vi "test_PhotonPoseEstimator_ClosestToCamera.vi"(8 "error in (no error)":errorcluster) -> (0 "error out":errorcluster, 3 "Test Passed":bool)   [LabVIEW 2019]
uses:
  <vilib>/Rock Robotics/WPI/ThirdParty/PhotonVisionLib/TypeDef/PhotonEstimatedRobotPoseType.ctl
  <vilib>/Rock Robotics/WPI/ThirdParty/JAS_Junk/TrajLib/TypeDef/POSE3D.ctl
  <vilib>/Rock Robotics/WPI/ThirdParty/JAS_Junk/TrajLib/TypeDef/TRANSLATION3D.ctl
  <vilib>/Rock Robotics/WPI/ThirdParty/JAS_Junk/TrajLib/TypeDef/ROTATION3D.ctl
  <vilib>/Rock Robotics/WPI/ThirdParty/JAS_Junk/TrajLib/TypeDef/QUATERNION.ctl
  <vilib>/Rock Robotics/WPI/ThirdParty/PhotonVisionLib/TypeDef/PhotonTrackedTargetType.ctl
  <vilib>/Rock Robotics/WPI/ThirdParty/PhotonVisionLib/TypeDef/TargetCornerType.ctl
  <vilib>/Rock Robotics/WPI/ThirdParty/JAS_Junk/TrajLib/TypeDef/TRANSFORM3D.ctl
  <vilib>/Rock Robotics/WPI/ThirdParty/PhotonVisionLib/Enum/PhotonPoseStrategy_ENUM.ctl
  <vilib>/Rock Robotics/WPI/ThirdParty/JAS_Junk/TrajLib/VI/Quaternion_New.vi
  <vilib>/Rock Robotics/WPI/ThirdParty/PhotonVisionLib/SubVI/PhotonTargetModel_New_AprilTag36H11.vi
  <vilib>/Rock Robotics/WPI/ThirdParty/JAS_Junk/TrajLib/VI/TimeInterpRotation2d_New.vi
  <vilib>/Rock Robotics/WPI/ThirdParty/JAS_Junk/TrajLib/VI/Transform3d_Equals.vi
  <vilib>/Rock Robotics/WPI/ThirdParty/PhotonVisionLib/SubVI/PhotonPoseEstimator_SetCamera.vi
  <vilib>/Rock Robotics/WPI/ThirdParty/PhotonVisionLib/SubVI/PhotonPoseEstimator_SetRobotToCameraTransform.vi
  <vilib>/Rock Robotics/WPI/ThirdParty/PhotonVisionLib/SubVI/PhotonPoseEstimator_SetLastPose.vi
  <vilib>/Rock Robotics/WPI/ThirdParty/PhotonVisionLib/SubVI/PhotonEstimatedRobotPose_GetAll.vi
  <vilib>/Rock Robotics/WPI/ThirdParty/JAS_Junk/TrajLib/VI/Pose3d_ToPose2d.vi
  <vilib>/Rock Robotics/WPI/ThirdParty/PhotonVisionLib/SubVI/PhotonPoseEstimator_GetEmptyPose.vi
  <vilib>/Rock Robotics/WPI/ThirdParty/PhotonVisionLib/SubVI/PhotonPoseEstimator_EstimateClosestToCameraHeightPose.vi
  <vilib>/Rock Robotics/WPI/ThirdParty/PhotonVisionLib/SubVI/PhotonPipelineResult_GetTimeStampSecs.vi
  <vilib>/Rock Robotics/WPI/ThirdParty/PhotonVisionLib/SubVI/PhotonPoseEstimator_Update_All.vi
  <vilib>/Rock Robotics/WPI/ThirdParty/PhotonVisionLib/SubVI/PhotonTargetModel_New_RectPlanar.vi
  <vilib>/Rock Robotics/WPI/ThirdParty/JAS_Junk/TrajLib/Conv_Inches_Meters.vi
  <vilib>/Rock Robotics/WPI/ThirdParty/JAS_Junk/TrajLib/VI/Transform3d_GetTranslation3d.vi
  <vilib>/Rock Robotics/WPI/ThirdParty/JAS_Junk/TrajLib/VI/Transform3d_GetRotation3d.vi
  <vilib>/Rock Robotics/WPI/ThirdParty/JAS_Junk/TrajLib/VI/Rotation3d_Equals.vi
  <vilib>/Rock Robotics/WPI/ThirdParty/JAS_Junk/TrajLib/VI/Translation3d_Equals.vi
  <vilib>/Rock Robotics/WPI/ThirdParty/JAS_Junk/TrajLib/VI/Pose3d_getTranslation3d.vi
  <vilib>/Rock Robotics/WPI/ThirdParty/JAS_Junk/TrajLib/VI/Pose3d_getRotation3d.vi
  <vilib>/Rock Robotics/WPI/ThirdParty/JAS_Junk/TrajLib/VI/Translation3d_ToTranslation2d.vi
  <vilib>/Rock Robotics/WPI/ThirdParty/JAS_Junk/TrajLib/VI/Rotation3d_ToRotation2d.vi
  <vilib>/Rock Robotics/WPI/ThirdParty/JAS_Junk/TrajLib/Pose2d_New_TRRO.vi
  <vilib>/Rock Robotics/WPI/ThirdParty/JAS_Junk/TrajLib/VI/Rotation3d_Create_AxisAngle.vi
  <vilib>/Rock Robotics/WPI/ThirdParty/JAS_Junk/TrajLib/VI/Pose3d_New.vi
  <vilib>/Rock Robotics/WPI/ThirdParty/PhotonVisionLib/SubVI/PhotonPipelineResult_HasTargets.vi
  <vilib>/Rock Robotics/WPI/ThirdParty/PhotonVisionLib/SubVI/PhotonEstimatedRobotPose_New.vi
  <vilib>/Rock Robotics/WPI/ThirdParty/PhotonVisionLib/SubVI/PhotonPipelineResult_GetTargets.vi
  <vilib>/Rock Robotics/WPI/ThirdParty/JAS_Junk/TrajLib/VI/AprilTagFieldLayout_GetTagPose.vi
  <vilib>/Rock Robotics/WPI/ThirdParty/PhotonVisionLib/SubVI/PhotonTrackedTarget_GetFiducialId.vi
  <vilib>/Rock Robotics/WPI/ThirdParty/PhotonVisionLib/SubVI/PhotonPoseEstimator_Strategy_closestToCameraHeight_calc.vi
  <vilib>/Rock Robotics/WPI/ThirdParty/PhotonVisionLib/SubVI/PhotonTrackedTarget_GetAltCameraToTarget.vi
  <vilib>/Rock Robotics/WPI/ThirdParty/PhotonVisionLib/SubVI/PhotonTrackedTarget_GetBestCameraToTarget.vi
  <vilib>/Rock Robotics/WPI/ThirdParty/PhotonVisionLib/SubVI/PhotonTrackedTarget_GetPoseAmbiguity.vi
  <vilib>/Rock Robotics/WPI/ThirdParty/PhotonVisionLib/SubVI/PhotonPoseEstimator_GetFieldTags.vi
  <vilib>/Rock Robotics/WPI/ThirdParty/PhotonVisionLib/SubVI/PhotonPoseEstimator_GetRobotToCameraTransform.vi
  <vilib>/Rock Robotics/WPI/ThirdParty/PhotonVisionLib/SubVI/PhotonPoseEstimator_GetHighestAmbiguity.vi
  <vilib>/Rock Robotics/WPI/ThirdParty/PhotonVisionLib/SubVI/PhotonPoseEstimator_EstimateLowestAmbiguityPose.vi
  <vilib>/Rock Robotics/WPI/ThirdParty/PhotonVisionLib/SubVI/PhotonPoseEstimator_EstimateClosestToReferencePose.vi
  <vilib>/Rock Robotics/WPI/ThirdParty/PhotonVisionLib/SubVI/PhotonPoseEstimator_GetReferencePose.vi
  <vilib>/Rock Robotics/WPI/ThirdParty/PhotonVisionLib/SubVI/PhotonPoseEstimator_GetLastPose.vi
  <vilib>/Rock Robotics/WPI/ThirdParty/PhotonVisionLib/SubVI/PhotonPoseEstimator_SetReferencePose.vi
  <vilib>/Rock Robotics/WPI/ThirdParty/PhotonVisionLib/SubVI/PhotonPoseEstimator_EstimateClosestToLastPose.vi
  <vilib>/Rock Robotics/WPI/ThirdParty/PhotonVisionLib/SubVI/PhotonPoseEstimator_EstimateAverageBestTargetsPose.vi
  <vilib>/Rock Robotics/WPI/ThirdParty/PhotonVisionLib/SubVI/PhotonPoseEstimator_EstimateMultiTagOnCoprocPose.vi
  <vilib>/Rock Robotics/WPI/ThirdParty/PhotonVisionLib/SubVI/PhotonPoseEstimator_EstimatePnpDistanceTrigSolvePose.vi
  <vilib>/Rock Robotics/WPI/ThirdParty/PhotonVisionLib/SubVI/PhotonPoseEstimator_Strategy_constrainedPnpStrategy.vi
  <vilib>/Rock Robotics/WPI/ThirdParty/PhotonVisionLib/SubVI/PhotonTargetModel_New.vi
  <vilib>/Rock Robotics/WPI/ThirdParty/JAS_Junk/TrajLib/VI/Rotation3d_GetQuaterion.vi
  <vilib>/Rock Robotics/WPI/ThirdParty/JAS_Junk/TrajLib/VI/Quaternion_Equals.vi
  <vilib>/Rock Robotics/WPI/ThirdParty/JAS_Junk/TrajLib/Translation2d_Create.vi
  <vilib>/Rock Robotics/WPI/ThirdParty/JAS_Junk/TrajLib/Rotation2d_CreateAngle.vi
  <vilib>/Rock Robotics/WPI/ThirdParty/JAS_Junk/TrajLib/VI/Rotation3d_GetXYZ.vi
  <vilib>/Rock Robotics/WPI/ThirdParty/JAS_Junk/TrajLib/VI/Rotation3d_Create_Default.vi
  <vilib>/Rock Robotics/WPI/ThirdParty/JAS_Junk/TrajLib/VI/Vector_Norm.vi
  <vilib>/Rock Robotics/WPI/ThirdParty/JAS_Junk/TrajLib/VecBuilder_ArrayBy1Fill.vi
  <vilib>/Rock Robotics/WPI/ThirdParty/JAS_Junk/TrajLib/VI/Pose3d_New_Trans3dRot3d.vi
  <vilib>/Rock Robotics/WPI/ThirdParty/JAS_Junk/TrajLib/VI/AprilTag_GetAll.vi
  <vilib>/Rock Robotics/WPI/ThirdParty/JAS_Junk/TrajLib/VI/Pose3d_RelativeTo.vi
  <vilib>/Rock Robotics/WPI/ThirdParty/JAS_Junk/TrajLib/VI/Pose3d_TransformBy.vi
  <vilib>/Rock Robotics/WPI/ThirdParty/JAS_Junk/TrajLib/VI/Transform3d_Inverse.vi
  <vilib>/Rock Robotics/WPI/ThirdParty/JAS_Junk/TrajLib/VI/Transform3d_GetXYZ.vi
  <vilib>/Rock Robotics/WPI/ThirdParty/JAS_Junk/TrajLib/VI/Pose3d_getXYZ.vi
  <vilib>/Rock Robotics/WPI/ThirdParty/JAS_Junk/TrajLib/Transform2d_Create_TransRot.vi
  <vilib>/Rock Robotics/WPI/ThirdParty/PhotonVisionLib/SubVI/PhotonPoseEstimator_Strategy_closestToReferencePose_calc.vi
  <vilib>/Rock Robotics/WPI/ThirdParty/PhotonVisionLib/SubVI/PhotonPoseEstimator_Strategy_averageBestTargets_calc.vi
  <vilib>/Rock Robotics/WPI/ThirdParty/JAS_Junk/TrajLib/VI/Rotation3d_Plus.vi
  <vilib>/Rock Robotics/WPI/ThirdParty/JAS_Junk/TrajLib/VI/Translation3d_Plus.vi
  <vilib>/Rock Robotics/WPI/ThirdParty/JAS_Junk/TrajLib/VI/Translation3d_Times.vi
  <vilib>/Rock Robotics/WPI/ThirdParty/JAS_Junk/TrajLib/VI/Rotation3d_Times.vi
  <vilib>/Rock Robotics/WPI/ThirdParty/JAS_Junk/TrajLib/VI/Translation3d_Create_Default.vi
  <vilib>/Rock Robotics/WPI/ThirdParty/JAS_Junk/TrajLib/VI/Pose3d_New_Default.vi
  <vilib>/Rock Robotics/WPI/ThirdParty/JAS_Junk/TrajLib/VI/Pose3d_Plus.vi
  <vilib>/Rock Robotics/WPI/ThirdParty/JAS_Junk/TrajLib/VI/AprilTagFieldLayout_GetOriginPosition.vi
  <vilib>/Rock Robotics/WPI/ThirdParty/PhotonVisionLib/SubVI/PhotonPipelineResult_GetMultiTagResult.vi
  <vilib>/Rock Robotics/WPI/ThirdParty/PhotonVisionLib/SubVI/PhotonPipelineResult_GetBestTarget.vi
  <vilib>/Rock Robotics/WPI/ThirdParty/PhotonVisionLib/SubVI/PhotonTrackedTarget_GetPitch.vi
  <vilib>/Rock Robotics/WPI/ThirdParty/PhotonVisionLib/SubVI/PhotonTrackedTarget_GetYaw.vi
  <vilib>/Rock Robotics/WPI/ThirdParty/JAS_Junk/TrajLib/Units_DegreesToRadians.vi
  <vilib>/Rock Robotics/WPI/ThirdParty/JAS_Junk/TrajLib/VI/Translation3d_GetNorm.vi
  <vilib>/Rock Robotics/WPI/ThirdParty/JAS_Junk/TrajLib/VI/Translation3d_Create_DistAng.vi
  <vilib>/Rock Robotics/WPI/ThirdParty/JAS_Junk/TrajLib/VI/Translation3d_RotateBy.vi
  <vilib>/Rock Robotics/WPI/ThirdParty/JAS_Junk/TrajLib/Translation2d_RotateBy.vi
  <vilib>/Rock Robotics/WPI/ThirdParty/JAS_Junk/TrajLib/Pose2d_getTranslation.vi
  <vilib>/Rock Robotics/WPI/ThirdParty/JAS_Junk/TrajLib/Translation2d_Plus.vi
  <vilib>/Rock Robotics/WPI/ThirdParty/JAS_Junk/TrajLib/Translation2d_UnaryMinus.vi
  <vilib>/Rock Robotics/WPI/ThirdParty/JAS_Junk/TrajLib/VI/Pose3d_New_Pose2d.vi
  <vilib>/Rock Robotics/WPI/ThirdParty/JAS_Junk/TrajLib/VI/TimeInterpRotation2d_GetSample.vi
  <vilib>/Rock Robotics/WPI/ThirdParty/PhotonVisionLib/SubVI/PhotonPoseEstimator_GetHeadingBuffer.vi
  <vilib>/Rock Robotics/WPI/ThirdParty/JAS_Junk/TrajLib/VI/Quaternion_Get_Vect.vi
  <vilib>/Rock Robotics/WPI/ThirdParty/JAS_Junk/TrajLib/VI/Quaternion_Get_W.vi
  <vilib>/Rock Robotics/WPI/ThirdParty/JAS_Junk/TrajLib/VI/Quaternion_Get_All.vi
  <vilib>/Rock Robotics/WPI/ThirdParty/JAS_Junk/TrajLib/VI/Quaternion_New_Default.vi
  <vilib>/Rock Robotics/WPI/ThirdParty/JAS_Junk/TrajLib/MatBuilder_Create.vi
  <vilib>/Rock Robotics/WPI/ThirdParty/JAS_Junk/TrajLib/VI/Transform3d_Create_Pose3dPose3d.vi
  <vilib>/Rock Robotics/WPI/ThirdParty/JAS_Junk/TrajLib/VI/Rotation3d_UnaryMinus.vi
  <vilib>/Rock Robotics/WPI/ThirdParty/JAS_Junk/TrajLib/VI/Translation3d_UnaryMinus.vi
  <vilib>/Rock Robotics/WPI/ThirdParty/JAS_Junk/TrajLib/VI/Translation3d_GetXYZ.vi
  <vilib>/Rock Robotics/WPI/ThirdParty/PhotonVisionLib/SubVI/PhotonPoseEstimator_CalcDifference.vi
  <vilib>/Rock Robotics/WPI/ThirdParty/JAS_Junk/TrajLib/VI/Rotation3d_RotateBy.vi
  <vilib>/Rock Robotics/WPI/ThirdParty/JAS_Junk/TrajLib/Conv_Deg_Radians.vi
  <vilib>/Rock Robotics/WPI/ThirdParty/JAS_Junk/TrajLib/VI/Quaternion_Times.vi
  <vilib>/Rock Robotics/WPI/ThirdParty/JAS_Junk/TrajLib/VI/Quaternion_Inverse.vi
  <vilib>/Rock Robotics/WPI/ThirdParty/JAS_Junk/TrajLib/Pose2d_getXYAngle.vi
  <vilib>/Rock Robotics/WPI/ThirdParty/JAS_Junk/TrajLib/Rotation2d_Interpolate.vi
  <vilib>/Rock Robotics/WPI/ThirdParty/JAS_Junk/TrajLib/VI/Translation3d_Minus.vi
  <vilib>/Rock Robotics/WPI/ThirdParty/JAS_Junk/TrajLib/VI/Rotation3d_Minus.vi
  <vilib>/Rock Robotics/WPI/ThirdParty/JAS_Junk/TrajLib/VI/Rotation3d_Create_Quaternion.vi
  <vilib>/Rock Robotics/WPI/ThirdParty/JAS_Junk/TrajLib/VI/Translation3d_GetDistance.vi
  <vilib>/Rock Robotics/WPI/ThirdParty/JAS_Junk/TrajLib/Rotation2d_Plus.vi
  <vilib>/Rock Robotics/WPI/ThirdParty/JAS_Junk/TrajLib/Rotation2d_Minus.vi
  <vilib>/Rock Robotics/WPI/ThirdParty/JAS_Junk/TrajLib/MathUtil_Clamp.vi
  <vilib>/Rock Robotics/WPI/ThirdParty/JAS_Junk/TrajLib/Rotation2d_Times.vi
  <vilib>/Rock Robotics/WPI/ThirdParty/JAS_Junk/TrajLib/VI/Quaternion_Normalize.vi
  <vilib>/Rock Robotics/WPI/ThirdParty/JAS_Junk/TrajLib/Rotation2d_RotateBy.vi
  <vilib>/Rock Robotics/WPI/ThirdParty/JAS_Junk/TrajLib/Rotation2d_UnaryMinus.vi
  <vilib>/Rock Robotics/WPI/ThirdParty/JAS_Junk/TrajLib/Rotation2d_CreateXY.vi
  <vilib>/Rock Robotics/WPI/ThirdParty/JAS_Junk/TrajLib/Util_CalcDist.vi
  <vilib>/Rock Robotics/WPI/ThirdParty/PhotonVisionLib/SubVI/PhotonVision_Globals.vi
  <vilib>/gmath/interp.llb/Search Ordered Table.vi
  <vilib>/Rock Robotics/WPI/ThirdParty/JAS_Junk/TrajLib/Trajectory_Library.lvlib
  <vilib>/Rock Robotics/WPI/ThirdParty/PhotonVisionLib/PhotonVisionLib.lvlib
panel:
  out "Test 2 Passed":bool
  out "Test 1 Passed":bool
  out "Pos Found":bool
  out "PhotonEstimatedRobotPose":T1={"EstimatedPose"={"Translation3d"={"X"=0.0, "Y"=0.0, "Z"=0.0}, "Rotation3d"={"Q_quaternion"={"R"=1.0, "V"=[0.0, 0.0, 0.0]}}}, "TimeStamp_Seconds"=0.0, "targetsUsed"=[], "Strategy"=enum."LOWEST_AMBIGUITY"} {"targetsUsed"."AltCameraToTarget"."TRANSLATION3D"."Z" format="%14.3f"; "targetsUsed"."AltCameraToTarget"."TRANSLATION3D"."Y" format="%14.3f"; "targetsUsed"."AltCameraToTarget"."TRANSLATION3D"."X" format="%14.3f"; "targetsUsed"."BestCameraToTarget"."TRANSLATION3D"."Z" format="%14.3f"; "targetsUsed"."BestCameraToTarget"."TRANSLATION3D"."Y" format="%14.3f"; "targetsUsed"."BestCameraToTarget"."TRANSLATION3D"."X" format="%14.3f"; "EstimatedPose"."Translation3d"."Z" format="%14.3f"; "EstimatedPose"."Translation3d"."Y" format="%14.3f"; "EstimatedPose"."Translation3d"."X" format="%14.3f"}
  out "Test 0 Passed":bool
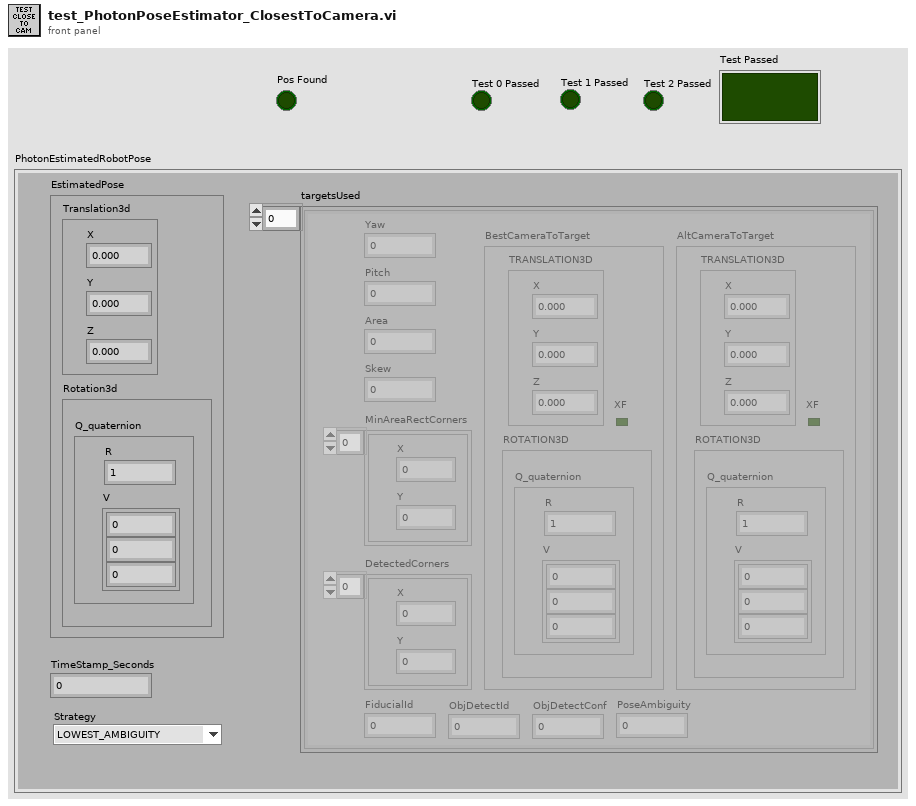
[diagram p1: front panel]
types:
  T1 = typedef "PhotonVisionLib.lvlib/PhotonEstimatedRobotPoseType.ctl" = cluster{"EstimatedPose":T2, "TimeStamp_Seconds":dbl, "targetsUsed":T6[], "Strategy":T9}
  T2 = typedef "Trajectory_Library.lvlib/POSE3D.ctl" = cluster{"Translation3d":T3, "Rotation3d":T4}
  T3 = typedef "Trajectory_Library.lvlib/TRANSLATION3D.ctl" = cluster{"X":dbl, "Y":dbl, "Z":dbl}
  T4 = typedef "Trajectory_Library.lvlib/ROTATION3D.ctl" = cluster{"Q_quaternion":T5}
  T5 = typedef "Trajectory_Library.lvlib/QUATERNION.ctl" = cluster{"R":dbl, "V":dbl[]}
  T6 = typedef "PhotonVisionLib.lvlib/PhotonTrackedTargetType.ctl" = cluster{"Yaw":dbl, "Pitch":dbl, "Area":dbl, "Skew":dbl, "MinAreaRectCorners":T7[], "BestCameraToTarget":T8, "FiducialId":i32, "AltCameraToTarget":T8, "PoseAmbiguity":dbl, "DetectedCorners":T7[], "ObjDetectId":i32, "ObjDetectConf":sgl}
  T7 = typedef "PhotonVisionLib.lvlib/TargetCornerType.ctl" = cluster{"X":dbl, "Y":dbl}
  T8 = typedef "Trajectory_Library.lvlib/TRANSFORM3D.ctl" = cluster{"TRANSLATION3D":T3, "ROTATION3D":T4, "XF":bool}
  T9 = typedef "PhotonVisionLib.lvlib/PhotonPoseStrategy_ENUM.ctl" = enum16{"LOWEST_AMBIGUITY", "CLOSEST_TO_CAMERA_HEIGHT", "CLOSEST_TO_REFERENCE_POSE", "CLOSEST_TO_LAST_POSE", "AVERAGE_BEST_TARGETS", "MULTI_TAG_PNP_ON_COPROCESSOR", "MULTI_TAG_PNP_ON_RIO", "PNP_DISTANCE_TRIG_SOLVE", "CONSTRAINED_SOLVEPNP"}
  T10 = typedef "Trajectory_Library.lvlib/AprilTagFieldLayout.ctl" = cluster{"AprilTagMap":map{i32, T11}, "FieldLength":dbl, "FieldWidth":dbl, "OriginPosition ":T12, "OriginPose3d":T2}
  T11 = typedef "Trajectory_Library.lvlib/AprilTag.ctl" = cluster{"ID":i32, "POSE3D":T2}
  T12 = typedef "Trajectory_Library.lvlib/AprilTagFieldLayoutOrignPosition_ENUM.ctl" = enum16{"kBlueAllianceWallRightSide,", "kRedAllianceWallRightSide,"}
  T13 = typedef "PhotonVisionLib.lvlib/PhotonPipelineMetadataType.ctl" = cluster{"CaptureTimestampMicros":i64, "PublishTimestampMicros":i64, "SequenceID":i64, "TimeSinceLastPong":i64}
  T14 = typedef "PhotonVisionLib.lvlib/PhotonPipelineResultType.ctl" = cluster{"Targets":T6[], "PhotonMultiTargetPNPResult":T15, "PhotonPipelineMetadata":T13}
  T15 = typedef "PhotonVisionLib.lvlib/PhotonMultiTargetPNPResultType.ctl" = cluster{"PhotonPNPResult":T16, "FiducialIDsUsed":i16[]}
  T16 = typedef "PhotonVisionLib.lvlib/PhotonPNPResultType.ctl" = cluster{"IsPresent":bool, "bestReprojErr":dbl, "altReprojErr":dbl, "ambiguity":dbl, "Best":T8, "Alt":T8}
  T17 = typedef "PhotonVisionLib.lvlib/PhotonPoseEstimator_Configuration.ctl" = cluster{"Primary Strategy":T9, "Camera":string, "Initial Pose":T2, "HighestAmbiguity":dbl, "RobotToCamera":T8, "FallBack Strategy":T9, "BaseNTName":string}
  T18 = typedef "PhotonVisionLib.lvlib/PhotonPoseEstimatorType.ctl" = cluster{"LastPose":T2, "ReferencePose":T2, "FieldTags":T10, "PrimaryStratety":T9, "Camera":string, "RobotToCamera":T8, "ReportedErrors":dbl[], "HighestAmbiguity":dbl, "MultiTagFallbackStrategy":T9, "PoseCacheTimeoutSec":dbl, "PhotonTargetModel":T19, "BaseNTName":string}
  T19 = typedef "PhotonVisionLib.lvlib/PhotonTargetModel.ctl" = cluster{"Vertices":T3[], "IsPlaner":bool, "IsSpherical":bool}
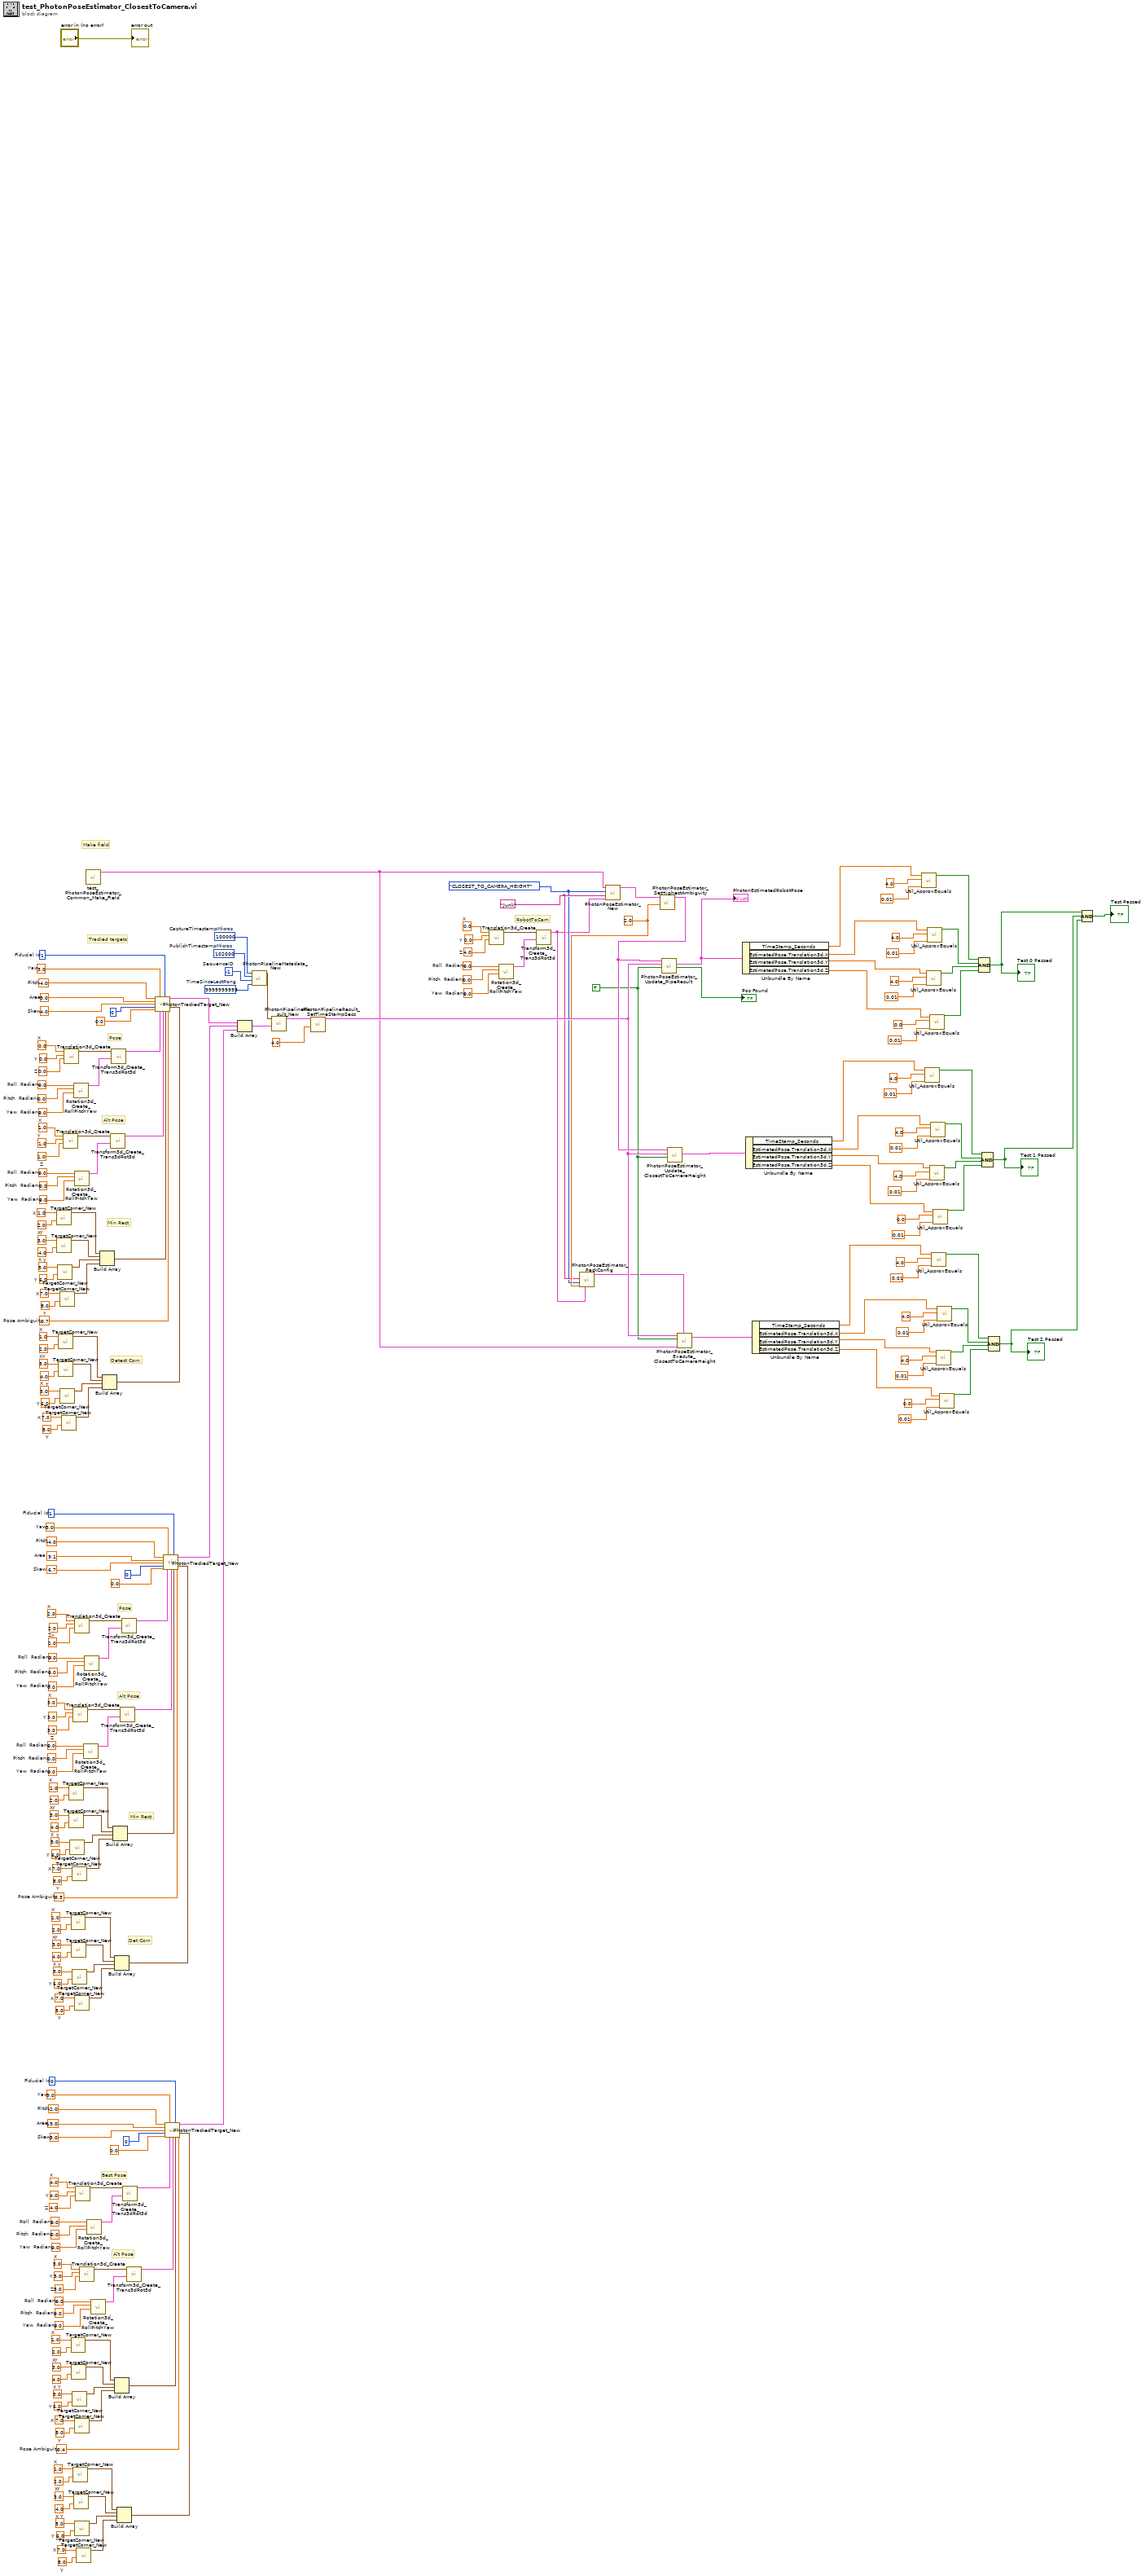
[diagram p0: block diagram]
diagram:
  w6 = 2.0 ("HighestAmbiguity")
  w54 = i64 100000  # CaptureTimestampMicros
  w55 = i64 102000  # PublishTimestampMicros
  w56 = i64 -1  # SequenceID
  w57 = i64 9999999999  # TimeSinceLastPong
  w43 = TRUE ("Has Results")
  w68 = 0.0  # Roll  Radians
  w67 = 0.0  # Pitch  Radians
  w66 = 0.0  # Yaw  Radians
  w71 = 4.0  # Z
  w70 = 0.0  # X
  w69 = 0.0  # Y
  w5 = "Junk" ("Camera")
  w4 = PhotonPoseStrategy_ENUM."CLOSEST_TO_CAMERA_HEIGHT" ("Strategy")
  w93 = 0.0  # Roll  Radians
  w92 = 0.0  # Pitch  Radians
  w91 = 0.0  # Yaw  Radians
  w96 = 4.0  # Z
  w95 = 4.0  # X
  w94 = 4.0  # Y
  w101 = 0.0  # Roll  Radians
  w100 = 0.0  # Pitch  Radians
  w99 = 0.0  # Yaw  Radians
  w104 = 5.0  # Z
  w103 = 5.0  # X
  w102 = 5.0  # Y
  w111 = 7.0  # X
  w112 = 8.0  # Y
  w113 = 5.0  # X
  w114 = 6.0  # Y
  w115 = 3.0  # X
  w116 = 4.0  # Y
  w117 = 1.0  # X
  w118 = 2.0  # Y
  w123 = 7.0  # X
  w124 = 8.0  # Y
  w125 = 5.0  # X
  w126 = 6.0  # Y
  w127 = 3.0  # X
  w128 = 4.0  # Y
  w129 = 1.0  # X
  w130 = 2.0  # Y
  w131 = -2.0  # Pitch
  w132 = 19.0  # Area
  w133 = 3.0  # Skew
  w134 = 0  # Fiducial Id
  w135 = 0.4  # Pose Ambiguity
  w136 = 9.0  # Yaw
  w143 = 0.0  # Roll  Radians
  w142 = 0.0  # Pitch  Radians
  w141 = 0.0  # Yaw  Radians
  w146 = 2.0  # Z
  w145 = 2.0  # X
  w144 = 2.0  # Y
  w151 = 0.0  # Roll  Radians
  w150 = 0.0  # Pitch  Radians
  w149 = 0.0  # Yaw  Radians
  w154 = 3.0  # Z
  w153 = 3.0  # X
  w152 = 3.0  # Y
  w161 = 7.0  # X
  w162 = 8.0  # Y
  w163 = 5.0  # X
  w164 = 6.0  # Y
  w165 = 3.0  # X
  w166 = 4.0  # Y
  w167 = 1.0  # X
  w168 = 2.0  # Y
  w173 = 7.0  # X
  w174 = 8.0  # Y
  w175 = 5.0  # X
  w176 = 6.0  # Y
  w177 = 3.0  # X
  w178 = 4.0  # Y
  w179 = 1.0  # X
  w180 = 2.0  # Y
  w181 = -4.0  # Pitch
  w182 = 9.1  # Area
  w183 = 6.7  # Skew
  w184 = 1  # Fiducial Id
  w185 = 0.3  # Pose Ambiguity
  w186 = 3.0  # Yaw
  w193 = 0.0  # Roll  Radians
  w192 = 0.0  # Pitch  Radians
  w191 = 0.0  # Yaw  Radians
  w196 = 0.0  # Z
  w195 = 0.0  # X
  w194 = 0.0  # Y
  w201 = 0.0  # Roll  Radians
  w200 = 0.0  # Pitch  Radians
  w199 = 0.0  # Yaw  Radians
  w204 = 1.0  # Z
  w203 = 1.0  # X
  w202 = 1.0  # Y
  w211 = 7.0  # X
  w212 = 8.0  # Y
  w213 = 5.0  # X
  w214 = 6.0  # Y
  w215 = 3.0  # X
  w216 = 4.0  # Y
  w217 = 1.0  # X
  w218 = 2.0  # Y
  w223 = 7.0  # X
  w224 = 8.0  # Y
  w225 = 5.0  # X
  w226 = 6.0  # Y
  w227 = 3.0  # X
  w228 = 4.0  # Y
  w229 = 1.0  # X
  w230 = 2.0  # Y
  w231 = -4.0  # Pitch
  w232 = 9.0  # Area
  w233 = 4.0  # Skew
  w234 = 1  # Fiducial Id
  w235 = 0.7  # Pose Ambiguity
  w236 = 3.0  # Yaw
  # "RobotToCam"
  # "Det Corn"
  # "Min Rect"
  # "Pose"
  # "Detect Corn"
  # "Min Rect"
  # "Tracked targets"
  # "Make field"
  # "Best Pose"
  # "Alt Pose"
  # "Alt Pose"
  # "Pose"
  # "Alt Pose"
  n1 = call <vilib>:"TargetCorner_New.vi"("Y"=w230, "X"=w229) -> ("TargetCorner"=w222:T7)  [unwired: 9 in]
  n2 = call <vilib>:"TargetCorner_New.vi"("Y"=w228, "X"=w227) -> ("TargetCorner"=w221:T7)  [unwired: 9 in]
  n3 = call <vilib>:"TargetCorner_New.vi"("Y"=w226, "X"=w225) -> ("TargetCorner"=w220:T7)  [unwired: 9 in]
  n4 = call <vilib>:"TargetCorner_New.vi"("Y"=w218, "X"=w217) -> ("TargetCorner"=w210:T7)  [unwired: 9 in]
  n5 = call <vilib>:"TargetCorner_New.vi"("Y"=w216, "X"=w215) -> ("TargetCorner"=w209:T7)  [unwired: 9 in]
  n6 = call <vilib>:"TargetCorner_New.vi"("Y"=w224, "X"=w223) -> ("TargetCorner"=w219:T7)  [unwired: 9 in]
  n7 = call <vilib>:"TargetCorner_New.vi"("Y"=w214, "X"=w213) -> ("TargetCorner"=w208:T7)  [unwired: 9 in]
  n8 = call <vilib>:"TargetCorner_New.vi"("Y"=w212, "X"=w211) -> ("TargetCorner"=w207:T7)  [unwired: 9 in]
  n9 = call <vilib>:"Translation3d_Create.vi"("Z"=w204, "Y"=w202, "X"=w203) -> ("TRANSLATION3D"=w198:T3)  [unwired: 8 in]
  n10 = call <vilib>:"Translation3d_Create.vi"("Z"=w196, "Y"=w194, "X"=w195) -> ("TRANSLATION3D"=w190:T3)  [unwired: 8 in]
  n11 = call <vilib>:"TargetCorner_New.vi"("Y"=w180, "X"=w179) -> ("TargetCorner"=w172:T7)  [unwired: 9 in]
  n12 = call <vilib>:"TargetCorner_New.vi"("Y"=w178, "X"=w177) -> ("TargetCorner"=w171:T7)  [unwired: 9 in]
  n13 = call <vilib>:"TargetCorner_New.vi"("Y"=w176, "X"=w175) -> ("TargetCorner"=w170:T7)  [unwired: 9 in]
  n14 = call <vilib>:"TargetCorner_New.vi"("Y"=w168, "X"=w167) -> ("TargetCorner"=w160:T7)  [unwired: 9 in]
  n15 = call <vilib>:"TargetCorner_New.vi"("Y"=w130, "X"=w129) -> ("TargetCorner"=w122:T7)  [unwired: 9 in]
  n16 = call <vilib>:"TargetCorner_New.vi"("Y"=w166, "X"=w165) -> ("TargetCorner"=w159:T7)  [unwired: 9 in]
  n17 = call <vilib>:"TargetCorner_New.vi"("Y"=w128, "X"=w127) -> ("TargetCorner"=w121:T7)  [unwired: 9 in]
  n18 = call <vilib>:"TargetCorner_New.vi"("Y"=w174, "X"=w173) -> ("TargetCorner"=w169:T7)  [unwired: 9 in]
  n19 = call <vilib>:"TargetCorner_New.vi"("Y"=w164, "X"=w163) -> ("TargetCorner"=w158:T7)  [unwired: 9 in]
  n20 = call <vilib>:"TargetCorner_New.vi"("Y"=w126, "X"=w125) -> ("TargetCorner"=w120:T7)  [unwired: 9 in]
  n21 = call <vilib>:"Translation3d_Create.vi"("Z"=w154, "Y"=w152, "X"=w153) -> ("TRANSLATION3D"=w148:T3)  [unwired: 8 in]
  n22 = call <vilib>:"TargetCorner_New.vi"("Y"=w118, "X"=w117) -> ("TargetCorner"=w110:T7)  [unwired: 9 in]
  n23 = call <vilib>:"Rotation3d_Create_RollPitchYaw.vi"("Yaw"=w191, "Pitch"=w192, "Roll"=w193) -> ("Rotation3d"=w189:T4)  [unwired: 8 in]
  n24 = call <vilib>:"TargetCorner_New.vi"("Y"=w116, "X"=w115) -> ("TargetCorner"=w109:T7)  [unwired: 9 in]
  n25 = call <vilib>:"Rotation3d_Create_RollPitchYaw.vi"("Yaw"=w199, "Pitch"=w200, "Roll"=w201) -> ("Rotation3d"=w197:T4)  [unwired: 8 in]
  n26 = call <vilib>:"Translation3d_Create.vi"("Z"=w146, "Y"=w144, "X"=w145) -> ("TRANSLATION3D"=w140:T3)  [unwired: 8 in]
  n27 = call <vilib>:"TargetCorner_New.vi"("Y"=w162, "X"=w161) -> ("TargetCorner"=w157:T7)  [unwired: 9 in]
  n28 = call <vilib>:"TargetCorner_New.vi"("Y"=w124, "X"=w123) -> ("TargetCorner"=w119:T7)  [unwired: 9 in]
  n29 = call <vilib>:"TargetCorner_New.vi"("Y"=w114, "X"=w113) -> ("TargetCorner"=w108:T7)  [unwired: 9 in]
  n30 = call <vilib>:"Translation3d_Create.vi"("Z"=w96, "Y"=w94, "X"=w95) -> ("TRANSLATION3D"=w90:T3)  [unwired: 8 in]
  n31 = call <vilib>:"TargetCorner_New.vi"("Y"=w112, "X"=w111) -> ("TargetCorner"=w107:T7)  [unwired: 9 in]
  n32 = call <vilib>:"Translation3d_Create.vi"("Z"=w104, "Y"=w102, "X"=w103) -> ("TRANSLATION3D"=w98:T3)  [unwired: 8 in]
  n33 = call <vilib>:"Rotation3d_Create_RollPitchYaw.vi"("Yaw"=w149, "Pitch"=w150, "Roll"=w151) -> ("Rotation3d"=w147:T4)  [unwired: 8 in]
  n34 = call <vilib>:"Rotation3d_Create_RollPitchYaw.vi"("Yaw"=w141, "Pitch"=w142, "Roll"=w143) -> ("Rotation3d"=w139:T4)  [unwired: 8 in]
  n35 = call "test_PhotonPoseEstimator_Common_Make_Field.vi"() -> ("AprilTagFieldLayout"=w42:T10)  [unwired: 11 in]
  n36 = call <vilib>:"Rotation3d_Create_RollPitchYaw.vi"("Yaw"=w91, "Pitch"=w92, "Roll"=w93) -> ("Rotation3d"=w89:T4)  [unwired: 8 in]
  n37 = call <vilib>:"Rotation3d_Create_RollPitchYaw.vi"("Yaw"=w99, "Pitch"=w100, "Roll"=w101) -> ("Rotation3d"=w97:T4)  [unwired: 8 in]
  n38 = Build Array(w222, w221, w220, w219) -> (w206:T7[])
  n39 = Build Array(w210, w209, w208, w207) -> (w205:T7[])
  n40 = call <vilib>:"Transform3d_Create_Trans3dRot3d.vi"("Rotation3d"=w197, "Translation3d"=w198) -> ("Transform3d"=w187:T8)  [unwired: 9 in]
  n41 = call <vilib>:"Transform3d_Create_Trans3dRot3d.vi"("Rotation3d"=w189, "Translation3d"=w190) -> ("Transform3d"=w188:T8)  [unwired: 9 in]
  n42 = Build Array(w172, w171, w170, w169) -> (w156:T7[])
  n43 = Build Array(w160, w159, w158, w157) -> (w155:T7[])
  n44 = Build Array(w122, w121, w120, w119) -> (w106:T7[])
  n45 = Build Array(w110, w109, w108, w107) -> (w105:T7[])
  n46 = call <vilib>:"Transform3d_Create_Trans3dRot3d.vi"("Rotation3d"=w147, "Translation3d"=w148) -> ("Transform3d"=w137:T8)  [unwired: 9 in]
  n47 = call <vilib>:"Transform3d_Create_Trans3dRot3d.vi"("Rotation3d"=w139, "Translation3d"=w140) -> ("Transform3d"=w138:T8)  [unwired: 9 in]
  n48 = call <vilib>:"Transform3d_Create_Trans3dRot3d.vi"("Rotation3d"=w89, "Translation3d"=w90) -> ("Transform3d"=w88:T8)  [unwired: 9 in]
  n49 = call <vilib>:"Transform3d_Create_Trans3dRot3d.vi"("Rotation3d"=w97, "Translation3d"=w98) -> ("Transform3d"=w87:T8)  [unwired: 9 in]
  n50 = call <vilib>:"PhotonTrackedTarget_New.vi"("Pitch"=w231, "Yaw"=w236, "Fiducial Id"=w234, "Area"=w232, "Skew"=w233, "ObjDetectId"=0, "DetectedCorners"=w205, "DetectObjConf"=sgl 0.0, "BestCameraToTarget"=w188, "AltCameraToTarget"=w187, "MinAreaRectCorners"=w206, "Pose Ambiguity"=w235) -> ("TrackedTarget"=w86:T6)  [unwired: 3 in]
  n51 = call <vilib>:"PhotonTrackedTarget_New.vi"("Pitch"=w181, "Yaw"=w186, "Fiducial Id"=w184, "Area"=w182, "Skew"=w183, "ObjDetectId"=0, "DetectedCorners"=w155, "DetectObjConf"=sgl 0.0, "BestCameraToTarget"=w138, "AltCameraToTarget"=w137, "MinAreaRectCorners"=w156, "Pose Ambiguity"=w185) -> ("TrackedTarget"=w85:T6)  [unwired: 3 in]
  n52 = call <vilib>:"PhotonTrackedTarget_New.vi"("Pitch"=w131, "Yaw"=w136, "Fiducial Id"=w134, "Area"=w132, "Skew"=w133, "ObjDetectId"=0, "DetectedCorners"=w105, "DetectObjConf"=sgl 0.0, "BestCameraToTarget"=w88, "AltCameraToTarget"=w87, "MinAreaRectCorners"=w106, "Pose Ambiguity"=w135) -> ("TrackedTarget"=w84:T6)  [unwired: 3 in]
  n53 = Build Array(w86, w85, w84) -> (w83:T6[])
  n54 = call <vilib>:"PhotonPipelineMetadata_New.vi"("TimeSinceLastPong"=w57, "SequenceID"=w56, "PublishTimestampMicros"=w55, "CaptureTimestampMicros"=w54) -> ("PhotonPipelineMetadata"=w53:T13)  [unwired: 7 in]
  n55 = call <vilib>:"PhotonPipelineResult_New.vi"("TrackedTargets"=w83, "Metadata"=w53) -> ("PhotonPipelineResult"=w82:T14)  [unwired: 9 in]
  n56 = call <vilib>:"PhotonPipelineResult_SetTimeStampSecs.vi"("TimeStampSec"=4.0, "PhotonPipelineResult"=w82) -> ("Out PhotonPipelineResult"=w44:T14)  [unwired: 9 in]
  n57 = call <vilib>:"Translation3d_Create.vi"("Z"=w71, "Y"=w69, "X"=w70) -> ("TRANSLATION3D"=w65:T3)  [unwired: 8 in]
  n58 = call <vilib>:"Rotation3d_Create_RollPitchYaw.vi"("Yaw"=w66, "Pitch"=w67, "Roll"=w68) -> ("Rotation3d"=w64:T4)  [unwired: 8 in]
  n59 = call <vilib>:"Transform3d_Create_Trans3dRot3d.vi"("Rotation3d"=w64, "Translation3d"=w65) -> ("Transform3d"=w3:T8)  [unwired: 9 in]
  n60 = call <vilib>:"PhotonPoseEstimator_PackConfig.vi"("RobotToCamera"=w3, "HighestAmbiguity"=w6, "PirmaryStrategy"=w4, "Camera"=w5) -> ("PoseEstimator_Configuration"=w7:T17)  [unwired: 7 in]
  n61 = call <vilib>:"PhotonPoseEstimator_New.vi"("RobotToCamera"=w3, "Camera"=w5, "Strategy"=w4, "AprilTagFieldLayout"=w42) -> ("PhotonPoseEstimator"=w46:T18)  [unwired: 7 in]
  n62 = call <vilib>:"PhotonPoseEstimator_SetHighestAmbiguity.vi"("HighestAmbiguity"=w6, "PhotonPoseEstimator"=w46) -> ("out PhotonPoseEstimator"=w45:T18)  [unwired: 9 in]
  n63 = call <vilib>:"PhotonPoseEstimator_Update_PipeResult.vi"("Has Results"=w43, "PipelineResult"=w44, "PhotonPoseEstimator"=w45) -> ("Pos Found"=→"Pos Found":bool, "PhotonEstimatedRobotPose"=w59:T1)  [unwired: 6 in, 1 out]
  "PhotonEstimatedRobotPose" <- w59
  n64 = call <vilib>:"PhotonPoseEstimator_Update_ClosestToCameraHeight.vi"("Has Results"=w43, "PipelineResult"=w44, "PhotonPoseEstimator"=w45) -> ("PhotonEstimatedRobotPose"=w25:T1)  [unwired: 6 in, 2 out]
  n65 = call <vilib>:"PhotonPoseEstimator_Execute_ClosestToCameraHeight.vi"("Configuration"=w7, "AprilTagFieldLayout"=w42, "PIpeline Has \nNew Results"=w43, "PipelineResult"=w44) -> ("PhotonEstimatedRobotPose"=w8:T1)  [unwired: 2 in, 5 out]
  n66 = Unbundle By Name(w59) -> ("TimeStamp_Seconds"=w60:dbl, "EstimatedPose.Translation3d.X"=w74:dbl, "EstimatedPose.Translation3d.Y"=w73:dbl, "EstimatedPose.Translation3d.Z"=w72:dbl)
  n67 = Unbundle By Name(w25) -> ("TimeStamp_Seconds"=w26:dbl, "EstimatedPose.Translation3d.X"=w32:dbl, "EstimatedPose.Translation3d.Y"=w31:dbl, "EstimatedPose.Translation3d.Z"=w30:dbl)
  n68 = Unbundle By Name(w8) -> ("TimeStamp_Seconds"=w9:dbl, "EstimatedPose.Translation3d.X"=w15:dbl, "EstimatedPose.Translation3d.Y"=w14:dbl, "EstimatedPose.Translation3d.Z"=w13:dbl)
  n69 = call <vilib>:"Util_ApproxEquals.vi"("Tolerance"=0.01, "Value 2"=4.0, "Value 1"=w60) -> ("ApproxEquals"=w61:bool)  [unwired: 8 in]
  n70 = call <vilib>:"Util_ApproxEquals.vi"("Tolerance"=0.01, "Value 2"=4.0, "Value 1"=w26) -> ("ApproxEquals"=w27:bool)  [unwired: 8 in]
  n71 = call <vilib>:"Util_ApproxEquals.vi"("Tolerance"=0.01, "Value 2"=4.0, "Value 1"=w73) -> ("ApproxEquals"=w76:bool)  [unwired: 8 in]
  n72 = call <vilib>:"Util_ApproxEquals.vi"("Tolerance"=0.01, "Value 2"=4.0, "Value 1"=w74) -> ("ApproxEquals"=w239:bool)  [unwired: 8 in]
  n73 = call <vilib>:"Util_ApproxEquals.vi"("Tolerance"=0.01, "Value 2"=0.0, "Value 1"=w72) -> ("ApproxEquals"=w75:bool)  [unwired: 8 in]
  n74 = call <vilib>:"Util_ApproxEquals.vi"("Tolerance"=0.01, "Value 2"=4.0, "Value 1"=w31) -> ("ApproxEquals"=w34:bool)  [unwired: 8 in]
  n75 = call <vilib>:"Util_ApproxEquals.vi"("Tolerance"=0.01, "Value 2"=4.0, "Value 1"=w32) -> ("ApproxEquals"=w39:bool)  [unwired: 8 in]
  n76 = call <vilib>:"Util_ApproxEquals.vi"("Tolerance"=0.01, "Value 2"=4.0, "Value 1"=w9) -> ("ApproxEquals"=w10:bool)  [unwired: 8 in]
  n77 = call <vilib>:"Util_ApproxEquals.vi"("Tolerance"=0.01, "Value 2"=0.0, "Value 1"=w30) -> ("ApproxEquals"=w33:bool)  [unwired: 8 in]
  n78 = call <vilib>:"Util_ApproxEquals.vi"("Tolerance"=0.01, "Value 2"=4.0, "Value 1"=w14) -> ("ApproxEquals"=w17:bool)  [unwired: 8 in]
  n79 = call <vilib>:"Util_ApproxEquals.vi"("Tolerance"=0.01, "Value 2"=4.0, "Value 1"=w15) -> ("ApproxEquals"=w22:bool)  [unwired: 8 in]
  n80 = call <vilib>:"Util_ApproxEquals.vi"("Tolerance"=0.01, "Value 2"=0.0, "Value 1"=w13) -> ("ApproxEquals"=w16:bool)  [unwired: 8 in]
  n81 = Compound Arithmetic op=AND(w61, w239, w76, w75) -> (w237:bool)
  "Test 0 Passed" <- w237
  n82 = Compound Arithmetic op=AND(w27, w39, w34, w33) -> (w2:bool)
  "Test 1 Passed" <- w2
  n83 = Compound Arithmetic op=AND(w10, w22, w17, w16) -> (w1:bool)
  "Test 2 Passed" <- w1
  n84 = Compound Arithmetic op=AND(w237, w2, w1) -> (→"Test Passed":bool)
  "error out" <- "error in (no error)"
